vi "FlatToRichcif_can_writer_cansub_RefreshDevices.vi"(5 "OutputClusterType":T1, 11 "InputCluster":T2) -> (3 "OutputCluster":T1)   [LabVIEW 2021, in "CanWriterCansub_client.lvlib"]
uses:
  CanWriterCansub_client.lvlib
  cif_can_writer_cansub_RefreshDevices_Flat.ctl
  cif_can_writer_cansub_RefreshDevices.ctl
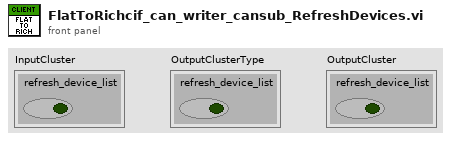
[diagram p1: front panel]
types:
  T1 = typedef "CanWriterCansub_client.lvlib/cif_can_writer_cansub_RefreshDevices.ctl" = cluster{"refresh_device_list":bool}
  T2 = typedef "CanWriterCansub_client.lvlib/cif_can_writer_cansub_RefreshDevices_Flat.ctl" = cluster{"refresh_device_list":bool}
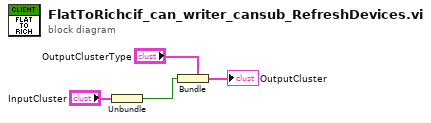
[diagram p0: block diagram]
diagram:
  n1 = Unbundle "Unbundle"("InputCluster") -> ("refresh_device_list"=w1:bool)
  n2 = Bundle "Bundle"(cluster="OutputClusterType", "refresh_device_list"=w1) -> (→"OutputCluster":T1)
